vi "First Token Index.vi"(8 "Tokens":string[](array[string]), 11 "String":string) -> (0 "token index":i32, 3 "String (dup)":string)   [LabVIEW 2021, in "Strings.lvlib"]
doc: "Returns the index of the first occurent of a token within a string (-2 if none is found)"
uses:
  <userlib>/_OpenG.lib/array/array.llb/Filter 1D Array (I32)__ogtk.vi
  Strings.lvlib
  <userlib>/_OpenG.lib/array/array.llb/openg_array.lvlib
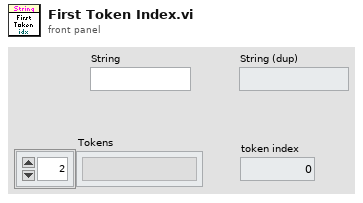
[diagram p1: front panel]
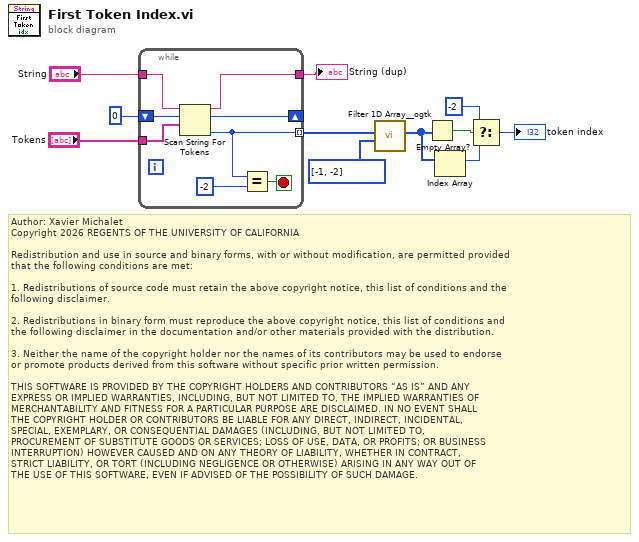
[diagram p0: block diagram]
diagram:
  # "Author: Xavier Michalet\nCopyright 2026 REGENTS OF THE UNIVERSITY OF CALIFORNIA\n\nRedistribution and use in source and binary forms, with or without modification, are permitted provided\nthat the following conditions are met:\n\n1. Redistributions of source code must retain the above copyright notice, this list of conditions and the\nfollowing disclaimer.\n\n2. Redistributions in binary form must reproduce the above copyright notice, this list of conditions and\nthe following disclaimer in the documentation and/or other materials provided with the distribution.\n\n3. Neither the name of the copyright holder nor the names of its contributors may be used to endorse \nor promote products derived from this software without specific prior written permission.\n\nTHIS SOFTWARE IS PROVIDED BY THE COPYRIGHT HOLDERS AND CONTRIBUTORS “AS IS” AND ANY \nEXPRESS OR IMPLIED WARRANTIES, INCLUDING, BUT NOT LIMITED TO, THE IMPLIED WARRANTIES OF\nMERCHANTABILITY AND FITNESS FOR A PARTICULAR PURPOSE ARE DISCLAIMED. IN NO EVENT SHALL\nTHE COPYRIGHT HOLDER OR CONTRIBUTORS BE LIABLE FOR ANY DIRECT, INDIRECT, INCIDENTAL, \nSPECIAL, EXEMPLARY, OR CONSEQUENTIAL DAMAGES (INCLUDING, BUT NOT LIMITED TO, \nPROCUREMENT OF SUBSTITUTE GOODS OR SERVICES; LOSS OF USE, DATA, OR PROFITS; OR BUSINESS\nINTERRUPTION) HOWEVER CAUSED AND ON ANY THEORY OF LIABILITY, WHETHER IN CONTRACT, \nSTRICT LIABILITY, OR TORT (INCLUDING NEGLIGENCE OR OTHERWISE) ARISING IN ANY WAY OUT OF\nTHE USE OF THIS SOFTWARE, EVEN IF ADVISED OF THE POSSIBILITY OF SUCH DAMAGE."
  n1 = while {
    tunnel: "Tokens" -> [w17]
    tunnel: "String" -> [w19]
    tunnel: [w18] -> w10
    shift-right: [w15] -> _
    shift-left: 0 ("offset") -> [w16]
    tunnel: [w12] -> w7 mode=indexing
    stop <- w13 stop-if-true
    n2 = Scan String For Tokens(7:w17, 8:w16, 9:w19) -> (0:w12:i32, 2:w15:i32, 3:w18:string)  [unwired: 3 in, 1 out]
    n3 = Equal?(x=w12, y=-2) -> (x = y?=w13:bool)
  }
  "String (dup)" <- w10
  n4 = call-poly <userlib>:"Filter 1D Array__ogtk.vi"("items to filter"=i32[] [-1, -2], "array"=w7) -> ("filtered array"=w5:i32[])  [unwired: 4 in, 1 out]
  n5 = Empty Array?(array=w5) -> (empty?=w6:bool)
  n6 = Index Array(array=w5) -> (element=w4:i32)  [unwired: 1 in]
  n7 = Select(t=-2, s=w6, f=w4) -> (s? t:f=→"token index":i32)
